vi "Read CE PSD Setting.vi"(8 "error in (no error)":errorcluster, 11 "SA Measurement in":refnum<class "SA Measurement.lvclass">) -> (0 "error out":errorcluster, 2 "CE PSD Setting":T1 {"Sweep Time(s)"."Time" format="%#_6p"; "RBW/VBW(Hz)"."VBW" format="%#_6p"; "RBW/VBW(Hz)"."RBW" format="%#_6p"; "Center and Span Frequency(Hz)"."Span" format="%#_6p"; "Center and Span Frequency(Hz)"."Center" format="%#_6p"; "Start/Stop Frequency(Hz)"."Stop" format="%#_6p"; "Start/Stop Frequency(Hz)"."Start" format="%#_6p"}, 3 "SA Measurement out":refnum<class "SA Measurement.lvclass">)   [LabVIEW 2023, in "Spectrum Analyzer.lvlib" / "SA Measurement.lvclass"]
uses:
  SA Measurement.lvclass
  SA Measurement.lvclass/SA Measurement.ctl
  TYPE DEFINITION/TYPE Start and Stop Frequency.ctl
  Spectrum Analyzer.lvlib
  TYPE DEFINITION/TYPE Center and Span Frequency.ctl
  TYPE DEFINITION/TYPE Reference Level and Atten Param.ctl
  TYPE DEFINITION/TYPE Y-axis Unit.ctl
  TYPE DEFINITION/TYPE Display Trace Mode Select.ctl
  TYPE DEFINITION/TYPE Detect Mode Select.ctl
  TYPE DEFINITION/TYPE Average Mode Select.ctl
  TYPE DEFINITION/SA Measurement Class/TYPE CE PSD Setting Parameter.ctl
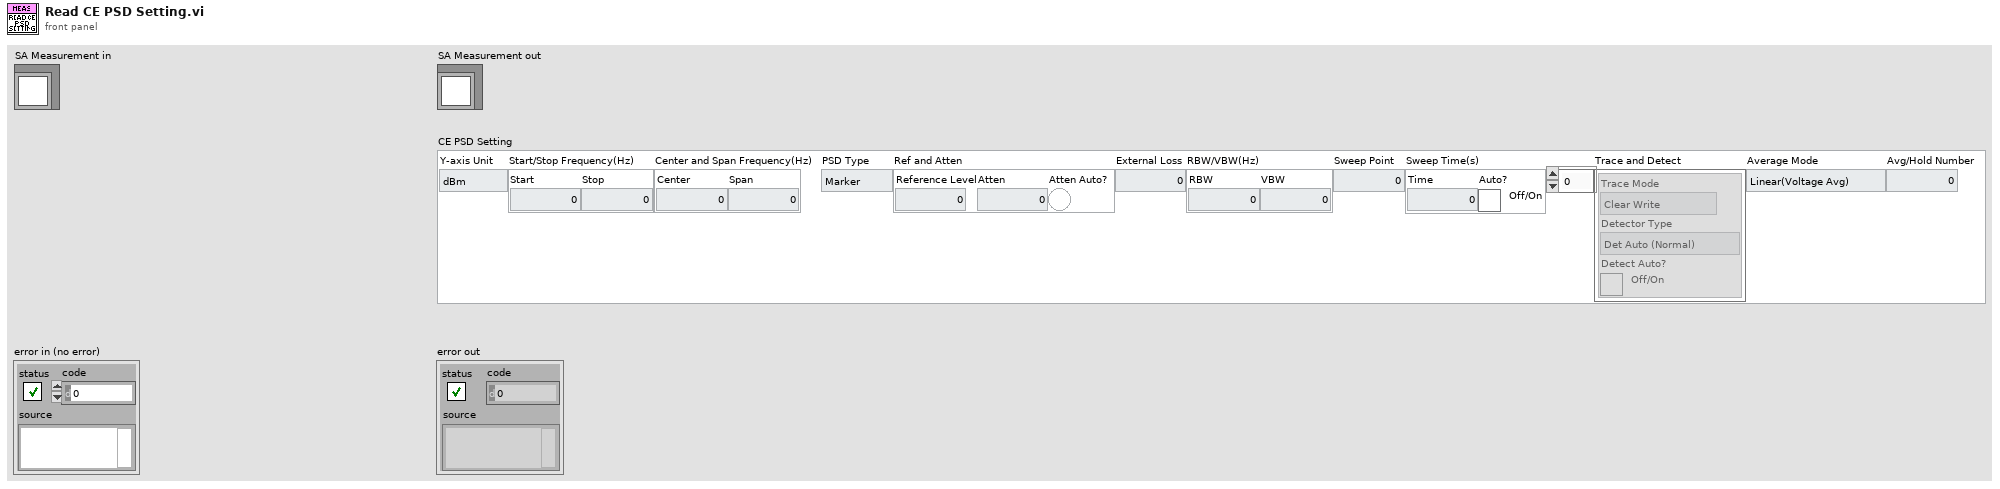
[diagram p1: front panel]
types:
  T1 = typedef "Spectrum Analyzer.lvlib/TYPE CE PSD Setting Parameter.ctl" = cluster{"Y-axis Unit":T2, "Start/Stop Frequency(Hz)":T3, "Center and Span Frequency(Hz)":T4, "PSD Type":enum16{"Marker", "Trace"}, "Ref and Atten":T5, "External Loss":dbl, "RBW/VBW(Hz)":cluster{"RBW":dbl, "VBW":dbl}, "Sweep Point":u32, "Sweep Time(s)":cluster{"Time":dbl, "Auto?":bool}, "Trace and Detect":cluster{"Trace Mode":T6, "Detector Type":T7, "Detect Auto?":bool}[], "Average Mode":T8, "Avg/Hold Number":u32}
  T2 = typedef "Spectrum Analyzer.lvlib/TYPE Y-axis Unit.ctl" = enum16{"dBm", "dBmV", "dBuV", "dBpW", "Volt", "Ampere", "Watt"}
  T3 = typedef "Spectrum Analyzer.lvlib/TYPE Start and Stop Frequency.ctl" = cluster{"Start":dbl, "Stop":dbl}
  T4 = typedef "Spectrum Analyzer.lvlib/TYPE Center and Span Frequency.ctl" = cluster{"Center":dbl, "Span":dbl}
  T5 = typedef "Spectrum Analyzer.lvlib/TYPE Reference Level and Atten Param.ctl" = cluster{"Reference Level":dbl, "Atten":i32, "Atten Auto?":bool}
  T6 = typedef "Spectrum Analyzer.lvlib/TYPE Display Trace Mode Select.ctl" = enum16{"Clear Write", "Max Hold", "Min Hold", "Average", "View"}
  T7 = typedef "Spectrum Analyzer.lvlib/TYPE Detect Mode Select.ctl" = enum16{"Det Auto (Normal)", "Auto Peak", "Positive Peak", "Negative Peak", "Sample", "RMS", "Average", "Quasipeak", "CISPR Average", "RMS Average"}
  T8 = typedef "Spectrum Analyzer.lvlib/TYPE Average Mode Select.ctl" = enum16{"Linear(Voltage Avg)", "Video(Log)", "Power"}
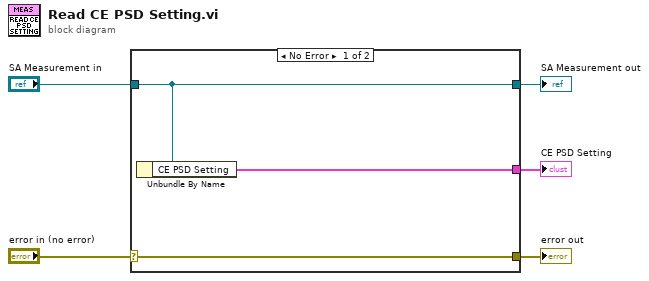
[diagram p0: block diagram]
diagram:
  n1 = case shown="No Error" "error in (no error)" {
    selector: "error in (no error)" -> [w8 w9]
    tunnel: [w8 w9] -> w4
    tunnel: [w7 w10] -> w2
    tunnel: "SA Measurement in" -> [w7 w10]
    tunnel: [w6 _] -> w1
    frame No Error {
      n2 = Unbundle By Name(w7) -> ("CE PSD Setting"=w6:T1)
    }
    frame Error {
    }
  }
  "error out" <- w4
  "SA Measurement out" <- w2
  "CE PSD Setting" <- w1
